vi "UseXctAnalysisDLL.vi"   [LabVIEW 2015]
uses:
  XCTAnalysis_DLL.dll
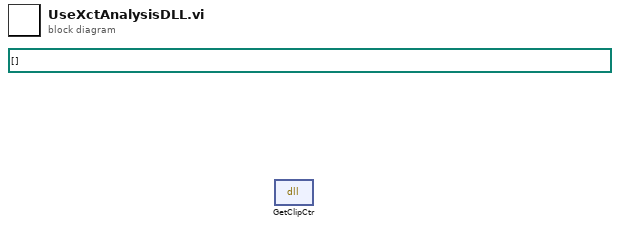
[diagram p0: block diagram]
diagram:
  (unwired) path[] []
  n1 = dll-call lib="C:/XctAnaDLL/Delphi/XCTAnalysis_DLL.dll" fn="GetClipCtr"() -> ()  [unwired: 4 in, 2 out]
